vi "Measurement Logic.vi"() -> ()   [LabVIEW 2022 SP3, in "Single Tone No Gen_Class D Amplifier.lvlib"]
uses:
  Single Tone No Gen_Class D Amplifier.lvlib
  Measurement Results.ctl
  shared/controls/units - snr.ctl
  shared/controls/audio controls.lvlib
  shared/controls/units - ratio.ctl
  shared/controls/units settings.ctl
  shared/controls/weighting filter.ctl
  shared/controls/highpass filter.ctl
  shared/controls/lowpass filter.ctl
  shared/controls/audio filter settings.ctl
  shared/controls/single tone audio measurement settings.ctl
  shared/analog input settings/Analog Input Settings.lvlib
  <vilib>/Waveform/WDTOps.llb/WDT Get Waveform Subset DBL.vi
  <vilib>/DAQmx/read.llb/DAQmx Read (Analog 1D Wfm NChan NSamp).vi
  <vilib>/DAQmx/configure/timing.llb/DAQmx Timing (Sample Clock).vi
  <vilib>/DAQmx/create/channels.llb/DAQmx Create Channel (AI-Voltage-Basic).vi
  shared/digital serial input settings/Digital Serial Input Settings.lvlib
  <vilib>/PDM Acquisition Toolkit/host/API/PDM Acquisition Toolkit.lvlib
  <vilib>/PDM Acquisition Toolkit/host/API/Public/Create Tasks/Create PCM Input Task.vi
  <vilib>/PDM Acquisition Toolkit/host/API/Public/Configure/Timing/Configure Timing - PCM Input Master.vi
  <vilib>/PDM Acquisition Toolkit/host/API/Public/Read/Read PCM Input Waveform.vi
  <vilib>/PDM Acquisition Toolkit/host/API/Public/Configure/PDM Channel/Configure Microphone Sensitivity FSPA - PCM Input Task.vi
  <vilib>/PDM Acquisition Toolkit/host/API/Public/Start/Start PCM Input Task.vi
  <vilib>/PDM Acquisition Toolkit/host/Classes/Tasks/PDM Tasks/Controls/Acquisition Mode.ctl
  <vilib>/PDM Acquisition Toolkit/host/Classes/Tasks/PDM Tasks/PDM Task.lvclass
  <vilib>/PDM Acquisition Toolkit/host/API/Public/Configure/Timing/Configure Timing - PCM Input Slave.vi
  <vilib>/PDM Acquisition Toolkit/shared/controls/clock mode.ctl
  <vilib>/PDM Acquisition Toolkit/shared/PDM Shared.lvlib
  Measurement Configuration.ctl
  <vilib>/Plug-In SDKs/Measurements/Measure Call Context/Measure Call Context.lvclass
panel:
  out "Spectrum":cluster{"x0":dbl, "dx":dbl, "magnitude":dbl[]}[](graph)
  out "Waveform Graph":waveform(dbl)[](graph)=[{"t0"=timestamp(3785336549.595634 s since 1904-01-01), "dt"=1.9531249997269942e-05, "Y"=array[12800 elements], "attributes"=variant("NI_ChannelName"=variant(string "PXI1Slot4/ai0"), "NI_UnitDescription"=variant(string "Volts"))}]
  out "measure call context out":refnum<class "Measure Call Context.lvclass">
  in  "measure call context in":refnum<class "Measure Call Context.lvclass">
  out "measurement results":T1={"channel names"=[], "frequency (Hz)"=[], "amplitude (Vrms)"=[], "amplitude (dBFS)"=[], "phase (deg)"=[], "SNR"=[], "THD+N"=[], "THD"=[], "dynamic range (dB)"=[], "gain"=[], "SFDR (dBc)"=[], "output power (W)"=[], "wfm - t0"=0.0, "wfm - dt"=1.9531249997269942e-05, "wfm - data"=array[12800 elements], "fft - f0"=0.0, "fft - df"=4.000000000559116, "fft - data"=array[6400 elements]}
  in  "measurement configuration":T2={"input configuration file"="PXI1Slot4/ai0", "digital channel list"="7821\\PCMo 8", "analog input channel"="", "min measurement cycles"=20, "min measurement time (s)"=0.1, "min settling cycles"=0, "min settling time (s)"=0.005, "band start"=20.0, "band stop"=20000.0, "weighting filter"=enum."Linear", "lowpass filter"=enum."No filter", "highpass filter"=enum."DC", "SNR units"=enum."dB", "THD+N units"=enum."dB", "THD units"=enum."dB", "gain units"=enum."dB", "expected amplitude (Vpk)"=2.0, "expected signal frequency"=51200.0, "amplitude reference (Vpk-pk)"=15.0, "load impedance"=4.0} {"load impedance" format="%#_13g"; "min settling time (s)" format="%#_6pHz"; "min measurement time (s)" format="%.0p"; "min measurement cycles" format="%0.2f"; "band start" format="%#_6pHz"}
  out "error out":errorcluster
  in  "error in":errorcluster
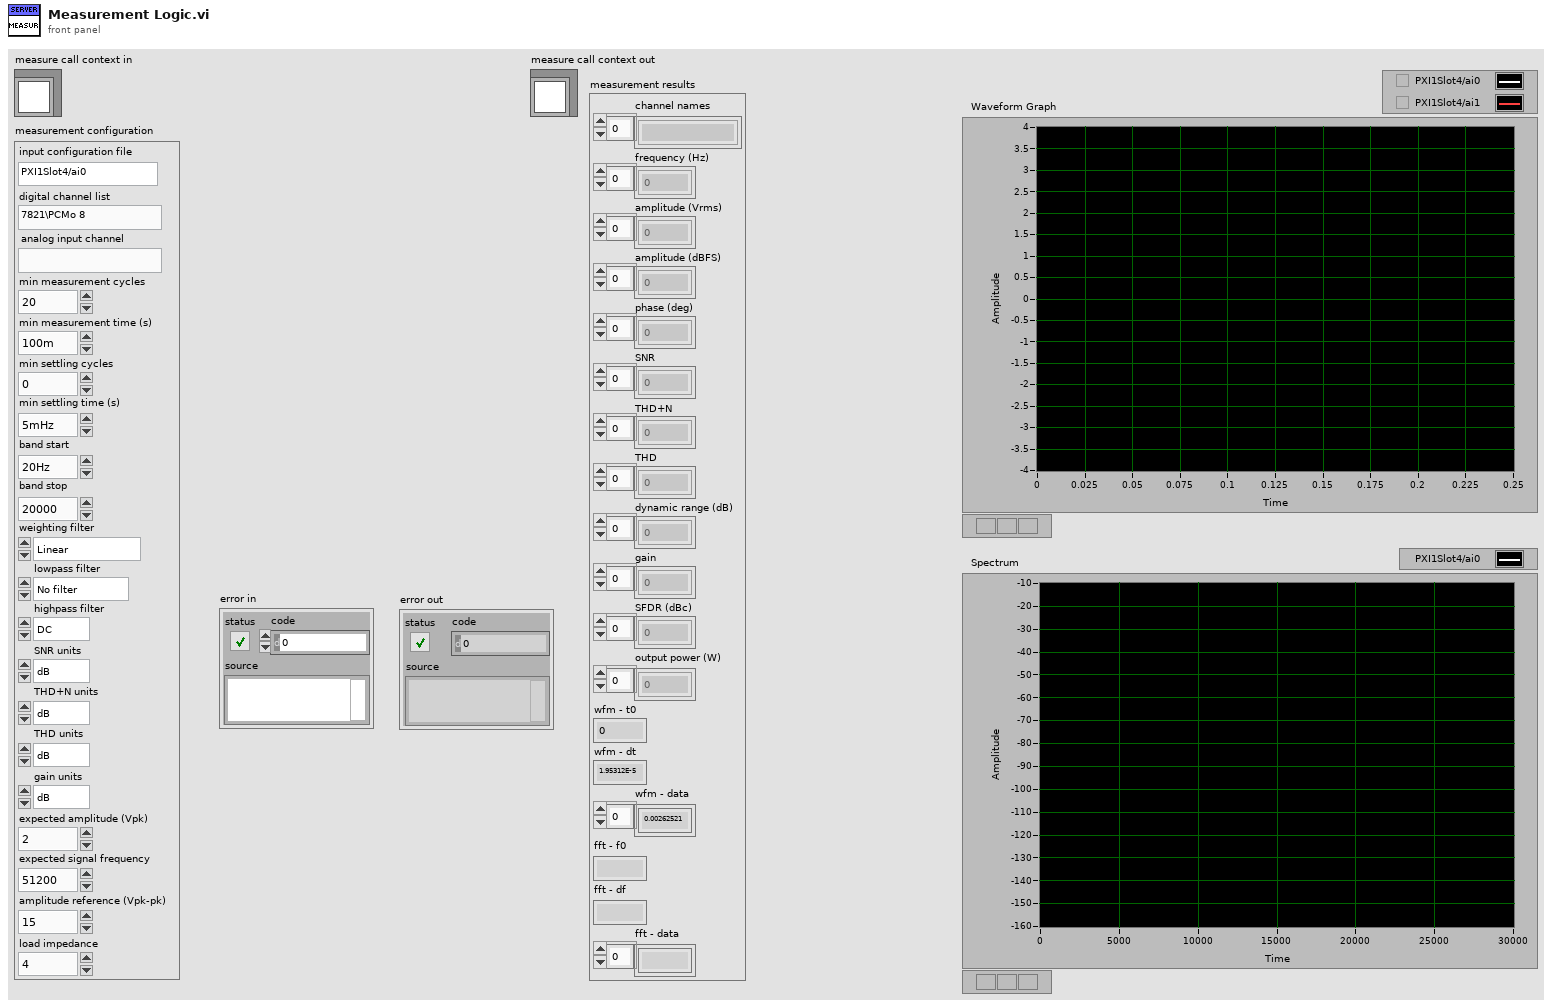
[diagram p1: front panel]
types:
  T1 = typedef "Single Tone No Gen_Class D Amplifier.lvlib/Measurement Results.ctl" = cluster{"channel names":string[], "frequency (Hz)":dbl[], "amplitude (Vrms)":dbl[], "amplitude (dBFS)":dbl[], "phase (deg)":dbl[], "SNR":dbl[], "THD+N":dbl[], "THD":dbl[], "dynamic range (dB)":dbl[], "gain":dbl[], "SFDR (dBc)":dbl[], "output power (W)":dbl[], "wfm - t0":dbl, "wfm - dt":dbl, "wfm - data":dbl[], "fft - f0":dbl, "fft - df":dbl, "fft - data":dbl[]}
  T2 = typedef "Single Tone No Gen_Class D Amplifier.lvlib/Measurement Configuration.ctl" = cluster{"input configuration file":string, "digital channel list":string, "analog input channel":string, "min measurement cycles":u32, "min measurement time (s)":dbl, "min settling cycles":u32, "min settling time (s)":dbl, "band start":dbl, "band stop":dbl, "weighting filter":T3, "lowpass filter":T4, "highpass filter":T5, "SNR units":T6, "THD+N units":T7, "THD units":T7, "gain units":T7, "expected amplitude (Vpk)":dbl, "expected signal frequency":dbl, "amplitude reference (Vpk-pk)":dbl, "load impedance":dbl}
  T3 = typedef "weighting filter.ctl" = enum32{"Linear", "A-weighting", "B-weighting", "C-weighting"}
  T4 = typedef "lowpass filter.ctl" = enum32{"No filter", "AES17 20kHz", "AES17 40kHz"}
  T5 = typedef "highpass filter.ctl" = enum32{"DC", "AC"}
  T6 = typedef "audio controls.lvlib/units - snr.ctl" = enum32{"dB", "x/y"}
  T7 = typedef "audio controls.lvlib/units - ratio.ctl" = enum32{"dB", "%", "x/y"}
  T8 = typedef "audio controls.lvlib/units settings.ctl" = cluster{"SNR units":T6, "THD+N units":T7, "THD units":T7, "gain units":T7}
  T9 = typedef "audio filter settings.ctl" = cluster{"weighting filter":T3, "highpass filter":T5, "lowpass filter ":T4}
  T10 = typedef "single tone audio measurement settings.ctl" = cluster{"Band start":dbl, "Band stop":dbl, "Amplitude":dbl, "Frequency":dbl, "Full scale range":dbl}
  T11 = typedef "acquisition type.ctl" = enum32{"Analog", "Digital Serial"}
  T12 = typedef "PDM Acquisition Class Library.lvlib/PDM Task.lvclass/Acquisition Mode.ctl" = enum16{"Finite", "Continuous"}
  T13 = typedef "PDM Shared.lvlib/clock mode.ctl" = enum16{"divided clock", "DDS"}
  T14 = typedef "AudioGenTypeDefs.lvlib/analog input settings.ctl" = cluster{"sample rate":dbl, "range":dbl, "terminal configuration":T15}
  T15 = typedef "AudioGenTypeDefs.lvlib/terminal configuration.ctl" = enum32{"Default", "RSE", "Differential", "Pseudodifferential"}
  T16 = typedef "digital serial input settings.ctl" = cluster{"number of channels":u32, "data justification":T17, "endianness":T18, "channel length":u32, "bit depth":u32, "frame clock rate":dbl, "bit clock edge sync":T19, "master clock source":T20, "master clock rate":dbl, "Logic Level":T21, "frame sync edge for channel 0":T19, "Channel 0 Offset":u32}
  T17 = typedef "PDM Shared.lvlib/PCM Data Justification.ctl" = enum16{"Left Justified", "Right Justified"}
  T18 = typedef "PDM Shared.lvlib/PCM Bit Endianness.ctl" = enum16{"MSB First", "LSB First"}
  T19 = typedef "PDM Shared.lvlib/Digital Edge.ctl" = enum8{"Rising", "Falling"}
  T20 = typedef "master clock source.ctl" = enum32{"Internal", "External"}
  T21 = typedef "PDM Acquisition Class Library.lvlib/DecoderSession.lvclass/Logic Levels.ctl" = enum16{"3.3 V", "1.8 V", "1.2 V"}
  T22 = typedef "PDM Shared.lvlib/PCM Data Format Configuration.ctl" = cluster{"Frame Sync Edge for Channel 0":T19, "Channel Count Per Frame":u8, "Channel Length":u16, "Bit Depth":u8, "Channel 0 Offset":u16, "Endianness":T18, "Data Justification":T17}
  T23 = typedef "PDM Shared.lvlib/PCM Frame Sync Control.ctl" = cluster{"Frame Length":u16, "Frame Sync Pulse Width":u16, "Bit Clock Edge  Sync":T19}
  T24 = typedef "PDM Acquisition Class Library.lvlib/PCM Input Task.lvclass/DVR PCM Input Task.ctl" = refnum<data-value>
  T25 = typedef "audio controls.lvlib/single tone audio measurements.ctl" = cluster{"channel":string, "frequency (Hz)":dbl, "amplitude (Vrms)":dbl, "amplitude (dBFS)":dbl, "phase (deg)":dbl, "SNR":dbl, "THD+N":dbl, "THD":dbl, "dynamic range (dB)":dbl, "gain":dbl, "SFDR (dBc)":dbl}
  T26 = typedef "audio controls.lvlib/single tone audio measurements (N chan).ctl" = cluster{"channel names":string[], "frequency (Hz)":dbl[], "amplitude (Vrms)":dbl[], "amplitude (dBFS)":dbl[], "phase (deg)":dbl[], "SNR":dbl[], "THD+N":dbl[], "THD":dbl[], "dynamic range (dB)":dbl[], "gain":dbl[], "SFDR (dBc)":dbl[]}
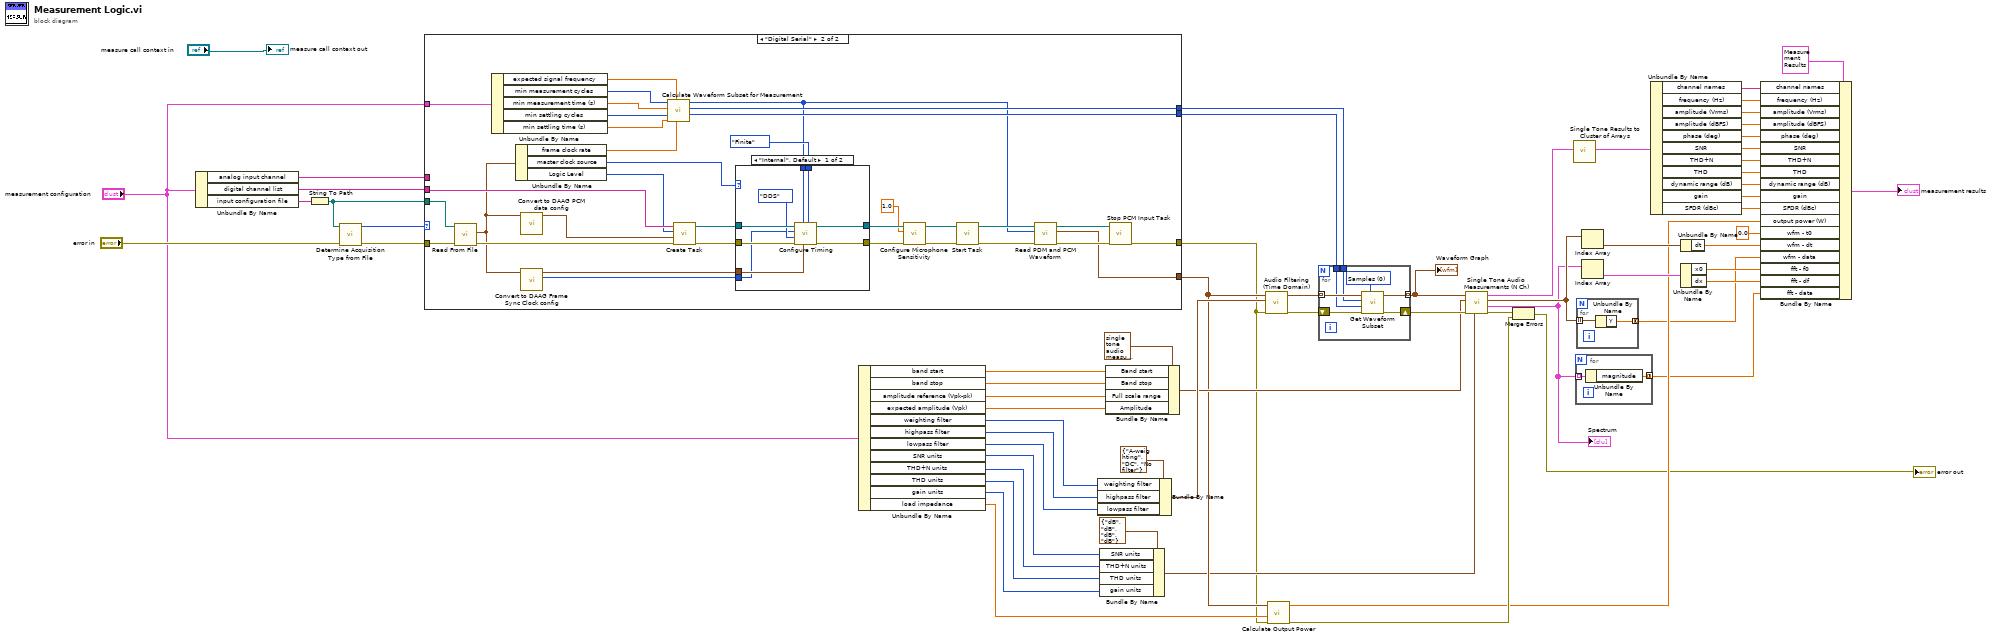
[diagram p0: block diagram]
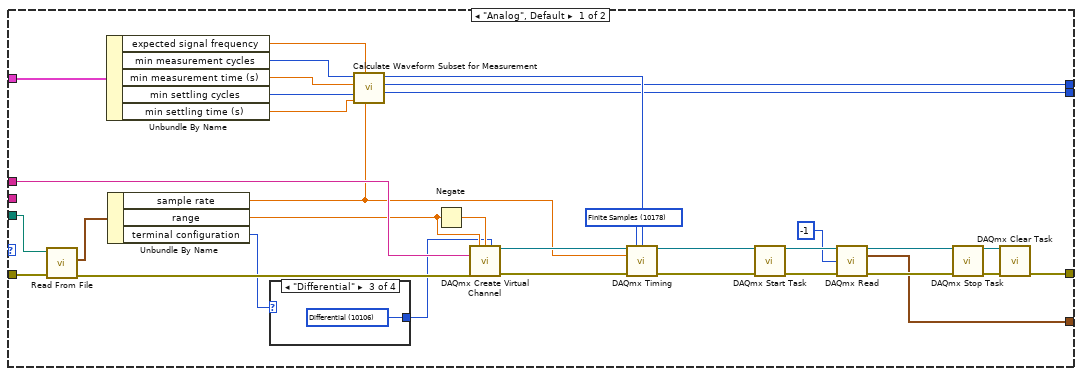
[diagram p2: hidden frame]
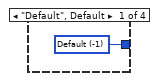
[diagram p3: hidden frame]
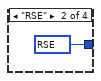
[diagram p4: hidden frame]
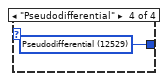
[diagram p5: hidden frame]
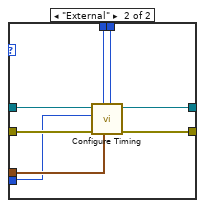
[diagram p6: hidden frame]
diagram:
  n1 = Unbundle By Name("measurement configuration") -> ("analog input channel"=w5:string, "digital channel list"=w4:string, "input configuration file"=w9:string)
  n2 = String To Path(string=w9) -> (path=w6:path)
  n3 = call "Determine Acquisition Type from File.vi"("error in (no error)"="error in", "cfg file"=w6) -> ("error out"=w8:errorcluster, "output type"=w7:T11)  [unwired: 8 in]
  n4 = case shown="\"Digital Serial\"" w7 {
    tunnel: [w86 w108] -> w45
    tunnel: [w85 w115] -> w37
    tunnel: w8 -> [w82 w135]
    tunnel: w6 -> [w83 w134]
    tunnel: w5 -> [w80 _]
    tunnel: w4 -> [_ w126]
    tunnel: "measurement configuration" -> [w71 w128]
    tunnel: [w68 w114] -> w2
    tunnel: [w67 w113] -> w1
    frame "Analog", Default {
      w88 = 10178 items=["Finite Samples"=10178, "Continuous Samples"=10123, "Hardware Timed Single Point"=12522] ("sample mode")
      n5 = call "Read From File.vi"("error in (no error)"=w82, "file path"=w83) -> ("error out"=w81:errorcluster, "analog input"=w79:T14)  [unwired: 7 in, 1 out]
      n6 = Unbundle By Name(w71) -> ("expected signal frequency"=w76:dbl, "min measurement cycles"=w72:u32, "min measurement time (s)"=w73:dbl, "min settling cycles"=w74:u32, "min settling time (s)"=w75:dbl)
      n7 = Unbundle By Name(w79) -> ("sample rate"=w70:dbl, "range"=w77:dbl, "terminal configuration"=w66:T15)
      n8 = case shown="\"Differential\"" w66 {
        tunnel: [w98 w99 w100 w101] -> w65
        frame "Default", Default {
          w98 = -1 items=["Default"=-1, "RSE"=10083, "NRSE"=10078, "Differential"=10106, "Pseudodifferential"=12529] ("input terminal configuration")
        }
        frame "RSE" {
          w99 = 10083 items=["Default"=-1, "RSE"=10083, "NRSE"=10078, "Differential"=10106, "Pseudodifferential"=12529] ("input terminal configuration")
        }
        frame "Differential" {
          w100 = 10106 items=["Default"=-1, "RSE"=10083, "NRSE"=10078, "Differential"=10106, "Pseudodifferential"=12529] ("input terminal configuration")
        }
        frame "Pseudodifferential" {
          w101 = 12529 items=["Default"=-1, "RSE"=10083, "NRSE"=10078, "Differential"=10106, "Pseudodifferential"=12529] ("input terminal configuration")
        }
      }
      n9 = call "Calculate Waveform Subset for Measurement.vi"("sampling rate"=w70, "signal frequency"=w76, "minimum settling duration"=w75, "minimum settling cycles"=w74, "minimum measurement duration"=w73, "minimum measurement cycles"=w72) -> ("duration (samples)"=w67:u32, "start (samples)"=w68:u32, "total acquisition (samples)"=w69:u32)  [unwired: 3 in]
      n10 = Negate(x=w77) -> (-x=w78:dbl)
      n11 = call-poly <vilib>:"DAQmx Create Virtual Channel.vi"("maximum value"=w77, "minimum value"=w78, "input terminal configuration"=w65, "physical channels"=w80, "error in"=w81) -> ("task out"=w96:refnum<k21>, "error out"=w97:errorcluster)  [unwired: 9 in]
      n12 = call-poly <vilib>:"DAQmx Timing.vi"("task/channels in"=w96, "sample mode"=w88, "samples per channel"=w69, "rate"=w70, "error in"=w97) -> ("task out"=w89:refnum<k21>, "error out"=w84:errorcluster)  [unwired: 9 in]
      n13 = call <vilib>:"DAQmx Start Task.vi"("task/channels in"=w89, "error in"=w84) -> ("task out"=w91:refnum<k21>, "error out"=w94:errorcluster)  [unwired: 12 in]
      n14 = call-poly <vilib>:"DAQmx Read.vi"("task/channels in"=w91, "number of samples per channel"=-1, "error in"=w94) -> ("task out"=w90:refnum<k21>, "data"=w86:waveform(dbl)[], "error out"=w93:errorcluster)  [unwired: 10 in]
      n15 = call <vilib>:"DAQmx Stop Task.vi"("task/channels in"=w90, "error in"=w93) -> ("task out"=w95:refnum<k21>, "error out"=w92:errorcluster)  [unwired: 12 in]
      n16 = call <vilib>:"DAQmx Clear Task.vi"("task in"=w95, "error in"=w92) -> ("error out"=w85:errorcluster)  [unwired: 13 in]
    }
    frame "Digital Serial" {
      n17 = call "Read From File.vi"("error in (no error)"=w135, "file path"=w134) -> ("error out"=w105:errorcluster, "digital serial input settings"=w104:T16)  [unwired: 7 in, 1 out]
      n18 = Unbundle By Name(w128) -> ("expected signal frequency"=w133:dbl, "min measurement cycles"=w129:u32, "min measurement time (s)"=w130:dbl, "min settling cycles"=w131:u32, "min settling time (s)"=w132:dbl)
      n19 = Unbundle By Name(w104) -> ("frame clock rate"=w127:dbl, "master clock source"=w111:T20, "Logic Level"=w106:T21)
      n20 = call "Convert to DAAG PCM data config.vi"("digital serial input settings"=w104) -> ("PCM data configuration"=w107:T22)  [unwired: 10 in]
      n21 = call "Convert to DAAG Frame Sync Clock config.vi"("digital serial input settings"=w104) -> ("Bit Clock rate"=w102:u32, "Frame Sync Clock Control"=w103:T23)  [unwired: 9 in]
      n22 = call "Calculate Waveform Subset for Measurement.vi"("sampling rate"=w127, "signal frequency"=w133, "minimum settling duration"=w132, "minimum settling cycles"=w131, "minimum measurement duration"=w130, "minimum measurement cycles"=w129) -> ("duration (samples)"=w113:u32, "start (samples)"=w114:u32, "total acquisition (samples)"=w109:u32)  [unwired: 3 in]
      n23 = call-poly <vilib>:"Create Task.vi"("error in"=w105, "PCM data configuration"=w107, "logic level"=w106, "channel list"=w126) -> ("error out"=w124:errorcluster, "PCM input task out"=w125:T24)  [unwired: 6 in]
      n24 = case shown="\"Internal\", Default" w111 {
        tunnel: w125 -> [w144 w152]
        tunnel: w124 -> [w143 w151]
        tunnel: [w142 w150] -> w119
        tunnel: [w141 w149] -> w118
        tunnel: w109 -> [w140 w148]
        tunnel: Acquisition_Mode."Finite" ("acquisition mode") -> [w139 w147]
        tunnel: w103 -> [w137 w146]
        tunnel: w102 -> [w136 w145]
        frame "Internal", Default {
          n25 = call-poly <vilib>:"Configure Timing.vi"("acquisition mode"=w139, "Frame Sync Clock Control"=w137, "number of words per channel"=w140, "error in"=w143, "clock mode"=clock_mode."DDS", "Bit Clock rate"=w136, "PCM input task in"=w144) -> ("error out"=w141:errorcluster, "PCM input task out"=w142:T24)  [unwired: 2 in, 1 out]
        }
        frame "External" {
          n26 = call-poly <vilib>:"Configure Timing.vi"("acquisition mode"=w147, "Frame Sync Clock Control"=w146, "number of words per channel"=w148, "error in"=w151, "Bit Clock rate"=w145, "PCM input task in"=w152) -> ("error out"=w149:errorcluster, "PCM input task out"=w150:T24)  [unwired: 4 in]
        }
      }
      n27 = call-poly <vilib>:"Configure Microphone Sensitivity.vi"("error in"=w118, "microphone sensitivity (FS/Pa)"=1.0, "PCM input task in"=w119) -> ("error out"=w116:errorcluster, "PCM input task out"=w117:T24)  [unwired: 7 in]
      n28 = call-poly <vilib>:"Start Task.vi"("error in"=w116, "PCM input task in"=w117) -> ("error out"=w120:errorcluster, "PCM input task out"=w121:T24)  [unwired: 8 in]
      n29 = call-poly <vilib>:"Read PDM and PCM Waveform.vi"("error in"=w120, "words per channel"=w109, "PCM input task In"=w121) -> ("error out"=w122:errorcluster, "PCM waveforms"=w108:waveform(dbl)[], "PCM input task out"=w123:T24)  [unwired: 3 in, 3 out]
      n30 = call <vilib>:"Stop PCM Input Task.vi"("error in"=w122, "PCM input task In"=w123) -> ("error out"=w115:errorcluster)  [unwired: 8 in, 1 out]
    }
  }
  n31 = Unbundle By Name("measurement configuration") -> ("band start"=w53:dbl, "band stop"=w52:dbl, "amplitude reference (Vpk-pk)"=w46:dbl, "expected amplitude (Vpk)"=w11:dbl, "weighting filter"=w12:T3, "highpass filter"=w50:T5, "lowpass filter"=w49:T4, "SNR units"=w41:T6, "THD+N units"=w40:T7, "THD units"=w39:T7, "gain units"=w38:T7, "load impedance"=w42:dbl)
  n32 = Bundle By Name(cluster=T9 {"weighting filter"=enum."A-weighting", "highpass filter"=enum."DC", "lowpass filter "=enum."No filter"} ("filter settings"), "weighting filter"=w12, "highpass filter"=w50, "lowpass filter"=w49) -> (w48:T9)
  n33 = Bundle By Name(cluster=T8 {"SNR units"=enum."dB", "THD+N units"=enum."dB", "THD units"=enum."dB", "gain units"=enum."dB"} ("units settings"), "SNR units"=w41, "THD+N units"=w40, "THD units"=w39, "gain units"=w38) -> (w43:T8)
  n34 = Bundle By Name(cluster=T10 {"Band start"=20.0, "Band stop"=20000.0, "Amplitude"=-1.0, "Frequency"=1000.0, "Full scale range"=15.0} ("measurement settings"), "Band start"=w53, "Band stop"=w52, "Full scale range"=w46, "Amplitude"=w11) -> (w47:T10)
  n35 = call "Audio Filtering (Time Domain).vi"("waveforms"=w45, "filter settings"=w48, "error in"=w37) -> ("time domain"=w57:waveform(dbl)[], "error out"=w58:errorcluster)  [unwired: 6 in]
  n36 = call "Calculate Output Power.vi"("error in (no error)"=w37, "load impedance"=w42, "waveforms"=w45) -> ("error out"=w59:errorcluster, "output power"=w18:dbl[])  [unwired: 7 in]
  n37 = for {
    tunnel: w57 -> [w159] mode=indexing
    tunnel: [w158] -> w36 mode=indexing
    shift-right: [w155] -> w56
    shift-left: w58 -> [w156]
    tunnel: w2 -> [w154]
    tunnel: w1 -> [w153]
    w157 = u16 0 items=["Samples", "Relative Time"] ("start/duration format")
    n38 = call-poly <vilib>:"Get Waveform Subset.vi"("start/duration format"=w157, "error in (no error)"=w156, "duration"=w153, "start samples/time"=w154, "waveform in"=w159) -> ("error out"=w155:errorcluster, "waveform out"=w158:waveform(dbl))  [unwired: 1 in, 2 out]
  }
  "Waveform Graph" <- w36
  n39 = call "Single Tone Audio Measurements (N Ch).vi"("units settings"=w43, "error in"=w56, "measurement settings"=w47, "waveforms"=w36) -> ("error out"=w55:errorcluster, "spectra"=w16:cluster{"x0":dbl, "dx":dbl, "magnitude":dbl[]}[], "waveforms"=w17:waveform(dbl)[], "results"=w31:T25[])  [unwired: 4 in]
  "Spectrum" <- w16
  n40 = Merge Errors(w55, w59) -> (→"error out":errorcluster)
  n41 = call "Single Tone Results to Cluster of Arrays.vi"("results"=w31) -> ("results (N chan)"=w30:T26)  [unwired: 10 in]
  n42 = for {
    tunnel: w16 -> [w161] mode=indexing
    tunnel: [w160] -> w15 mode=concatenating
    n43 = Unbundle By Name(w161) -> ("magnitude"=w160:dbl[])
  }
  n44 = for {
    tunnel: w17 -> [w163] mode=indexing
    tunnel: [w162] -> w14 mode=concatenating
    n45 = Unbundle By Name(w163) -> ("Y"=w162:dbl[])
  }
  n46 = Index Array(array=w17) -> (element=w35:waveform(dbl))  [unwired: 1 in]
  n47 = Index Array(array=w16) -> (element=w34:cluster{"x0":dbl, "dx":dbl, "magnitude":dbl[]})  [unwired: 1 in]
  n48 = Unbundle By Name(w30) -> ("channel names"=w29:string[], "frequency (Hz)"=w28:dbl[], "amplitude (Vrms)"=w27:dbl[], "amplitude (dBFS)"=w26:dbl[], "phase (deg)"=w25:dbl[], "SNR"=w24:dbl[], "THD+N"=w23:dbl[], "THD"=w22:dbl[], "dynamic range (dB)"=w21:dbl[], "gain"=w20:dbl[], "SFDR (dBc)"=w19:dbl[])
  n49 = Unbundle By Name(w35) -> ("dt"=w63:dbl)
  n50 = Unbundle By Name(w34) -> ("x0"=w62:dbl, "dx"=w61:dbl)
  n51 = Bundle By Name(cluster=T1 {"channel names"=[], "frequency (Hz)"=[], "amplitude (Vrms)"=[], "amplitude (dBFS)"=[], "phase (deg)"=[], "SNR"=[], "THD+N"=[], "THD"=[], "dynamic range (dB)"=[], "gain"=[], "SFDR (dBc)"=[], "output power (W)"=[], "wfm - t0"=0.0, "wfm - dt"=0.0, "wfm - data"=[], "fft - f0"=0.0, "fft - df"=0.0, "fft - data"=[]} ("Measurement Results"), "channel names"=w29, "frequency (Hz)"=w28, "amplitude (Vrms)"=w27, "amplitude (dBFS)"=w26, "phase (deg)"=w25, "SNR"=w24, "THD+N"=w23, "THD"=w22, "dynamic range (dB)"=w21, "gain"=w20, "SFDR (dBc)"=w19, "output power (W)"=w18, "wfm - t0"=0.0, "wfm - dt"=w63, "wfm - data"=w14, "fft - f0"=w62, "fft - df"=w61, "fft - data"=w15) -> (→"measurement results":T1)
  "measure call context out" <- "measure call context in"
